vi "Test_Bench_2.vi"() -> ()   [LabVIEW 2024]
uses:
  GPIB_Address.vi
panel:
  out "for loop repeat":i32
  in  "address string":string="23"
  out "Unaveraged data":string[][](array[string])
  in  "file path (use dialog) 2":path=path "C:/Users/Crawford Group/Desktop/Angelo/NMR/DATA/Unaveraged&TimeStamp.txt"
  in  "file path (use dialog)":path=path "C:/Users/Crawford Group/Desktop/Angelo/NMR/DATA/DATA.txt"
  out "x <= y?":bool
  out "x*y 2":i32
  out "x*y":dbl
  out "Array":string[][](array[string])
  in  "Number of T- Set Sweeps":i32
  # "DATA"
  # "Unaveraged"
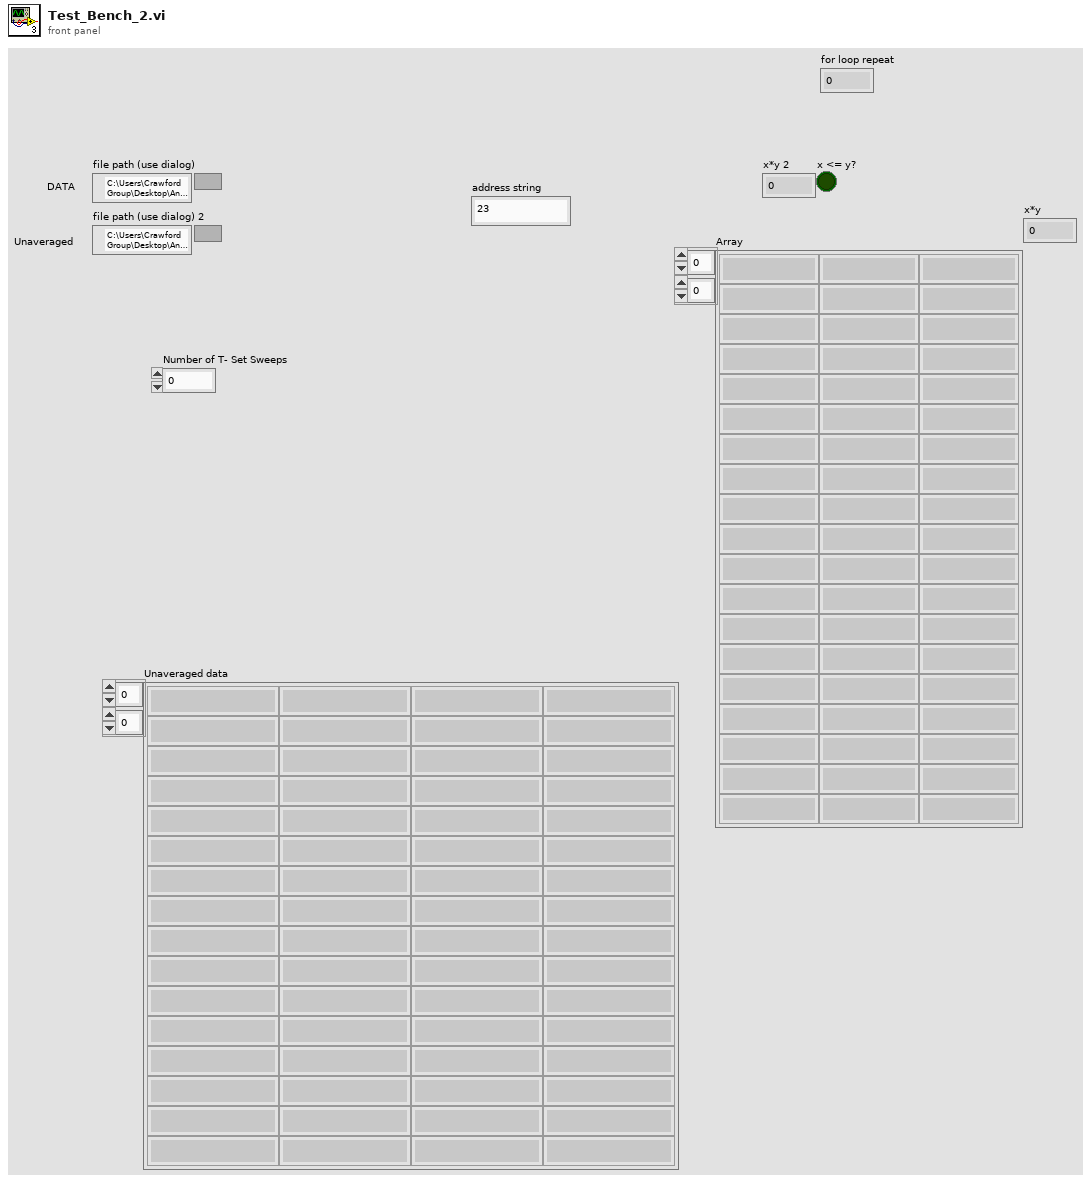
[diagram p1: front panel]
types:
  T1 = enum16{"open", "replace", "create", "open or create", "replace or create", "replace or create with confirmation"}
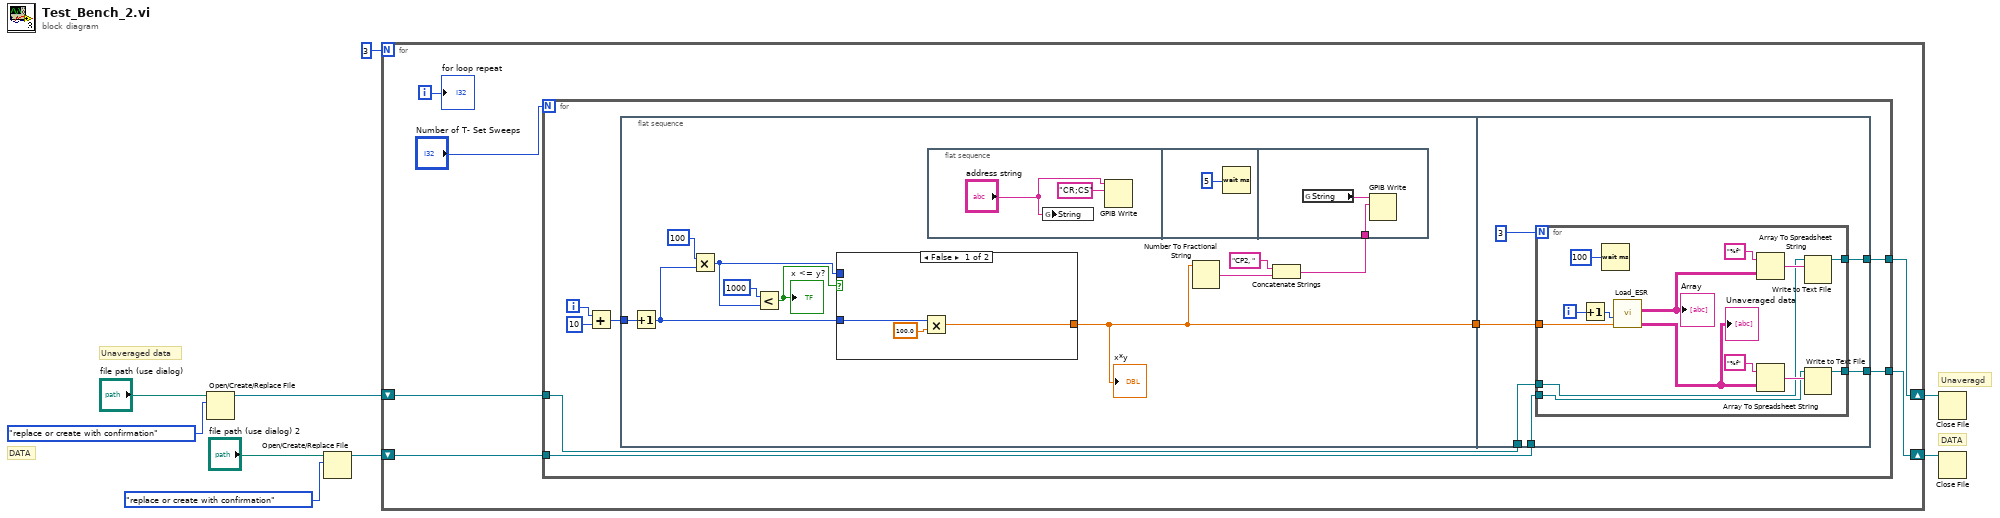
[diagram p0: block diagram]
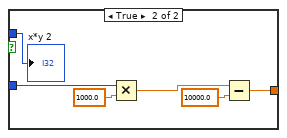
[diagram p2: hidden frame]
diagram:
  # "DATA"
  # "Unaveragd"
  # "Unaveraged data"
  # "DATA"
  n1 = Open/Create/Replace File(file path (use dialog)="file path (use dialog)", operation (0:open)=T1."replace or create with confirmation") -> (refnum out=w3:refnum<file>)  [unwired: 4 in, 2 out]
  n2 = Open/Create/Replace File(file path (use dialog)="file path (use dialog) 2", operation (0:open)=T1."replace or create with confirmation") -> (refnum out=w2:refnum<file>)  [unwired: 4 in, 2 out]
  n3 = for {
    N: 3 -> [_]
    shift-right: [w14] -> w8
    shift-left: w3 -> [w12]
    shift-right: [w13] -> w7
    shift-left: w2 -> [w11]
    i -> [w10]
    n4 = for {
      N: "Number of T- Set Sweeps" -> [_]
      tunnel: [w22] -> w14
      tunnel: [w21] -> w13
      tunnel: w12 -> [w20]
      tunnel: w11 -> [w19]
      i -> [w16]
      n5 = Add(x=w16, y=10) -> (x+y=w17:i32)
      n6 = flat-sequence {
        tunnel: w17 -> [w29]
        tunnel: [w30] -> w23
        tunnel: w23 -> [w52]
        tunnel: [w51] -> w22
        tunnel: [w50] -> w21
        tunnel: w20 -> [w49]
        tunnel: w19 -> [w48]
        frame #0 {
          n7 = Increment(x=w29) -> (x+1=w28:i32)
          n8 = Multiply(x=100, y=w28) -> (x*y=w24:i32)
          n9 = Less?(x=1000, y=w24) -> (x < y?=w25:bool)
          "x <= y?" <- w25
          n10 = case shown="False" w25 {
            tunnel: [w35 w38] -> w30
            tunnel: w28 -> [w34 w41]
            tunnel: w24 -> [_ w37]
            frame False {
              n11 = Multiply(x=w34, y=100.0) -> (x*y=w35:dbl)
            }
            frame True {
              n12 = Multiply(x=w41, y=1000.0) -> (x*y=w40:dbl)
              n13 = Subtract(x=w40, y=10000.0) -> (x-y=w38:dbl)
              "x*y 2" <- w37
            }
          }
          "x*y" <- w30
          n14 = flat-sequence {
            tunnel: w31 -> [w47]
            frame #0 {
              n15 = global write "GPIB_Address.vi" "String"("address string") -> ()
              n16 = GPIB Write(0:"address string", 1:"CR;CS" ("data")) -> ()  [unwired: 3 in, 2 out]
            }
            frame #1 {
              n17 = Wait (ms)(milliseconds to wait=u32 5) -> ()  [unwired: 1 out]
            }
            frame #2 {
              n18 = global read "GPIB_Address.vi" "String"() -> (w46:string)
              n19 = GPIB Write(0:w46, 1:w47) -> ()  [unwired: 3 in, 2 out]
            }
          }
          n20 = Number To Fractional String(number=w30) -> (F-format string=w32:string)  [unwired: 3 in]
          n21 = Concatenate Strings("CP2, " ("string"), w32) -> (w31:string)
        }
        frame #1 {
          n22 = for {
            N: 3 -> [_]
            tunnel: w52 -> [w67]
            tunnel: [w58] -> w51
            tunnel: [w57] -> w50
            tunnel: w49 -> [w56]
            tunnel: w48 -> [w55]
            i -> [w66]
            n23 = Increment(x=w66) -> (x+1=w65:i32)
            n24 = Wait (ms)(milliseconds to wait=u32 100) -> ()  [unwired: 1 out]
            n25 = call "Load_ESR.vi"("Tset setting"=w67, "N per point"=w65) -> ("Unaveraged data"=w59:string[][], "Data"=w62:string[][])  [unwired: 7 in, 1 out]
            "Array" <- w62
            "Unaveraged data" <- w59
            n26 = Array To Spreadsheet String(array=w62, 3:"%f" ("format string")) -> (spreadsheet string=w64:string)  [unwired: 1 in]
            n27 = Array To Spreadsheet String(array=w59, 3:"%f" ("format string")) -> (spreadsheet string=w61:string)  [unwired: 1 in]
            n28 = Write to Text File(file (use dialog)=w56, text=w64) -> (refnum out=w58:refnum<file>)  [unwired: 2 in, 2 out]
            n29 = Write to Text File(file (use dialog)=w55, text=w61) -> (refnum out=w57:refnum<file>)  [unwired: 2 in, 2 out]
          }
        }
      }
    }
    "for loop repeat" <- w10
  }
  n30 = Close File(refnum=w8) -> ()  [unwired: 1 in, 2 out]
  n31 = Close File(refnum=w7) -> ()  [unwired: 1 in, 2 out]
